vi "[ce low] Find All Min & Max of f(x).vi"(5 "# points":u32=1000, 6 "accuracy":dbl=1e-08 format="%.2e", 7 "VC Handle":T1=-1, 8 "error in":errorcluster, 9 "formula info":cluster{"formula":string, "x-variable":string}={"formula"="", "x-variable"="t"}, 10 "end":dbl=1.0 format="%.2f", 11 "start":dbl format="%.2f") -> (0 "error out":errorcluster, 2 "minima":cluster{"x":dbl[], "f(x)":dbl[]} {"f(x)" format="%.2f"; "x" format="%.2f"}, 3 "maxima":cluster{"x":dbl[], "f(x)":dbl[]} {"f(x)" format="%.2f"; "x" format="%.2f"})   [LabVIEW 2021]
doc: "::: CalcExpress Toolkit :::\nCopyright (c) 2000-2026 Konstantin Shifershteyn. All rights reserved."
uses:
  cetypes.llb/VarMan Variable Context Handle.ctl
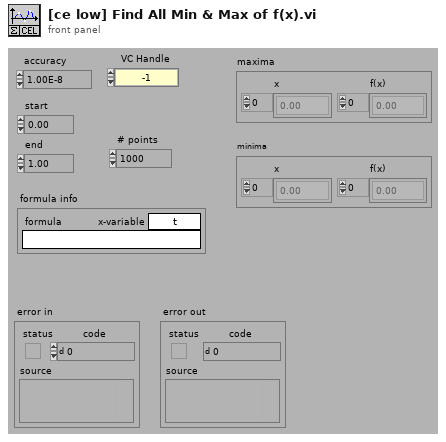
[diagram p1: front panel]
types:
  T1 = typedef "VarMan Variable Context Handle.ctl" = i32
  T2 = enum16{"create", "destroy", "set value", "get value"}
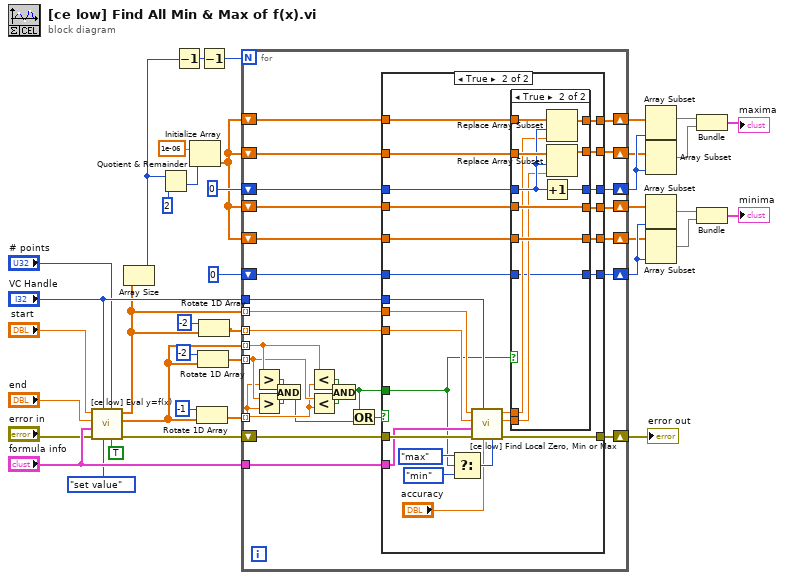
[diagram p0: block diagram]
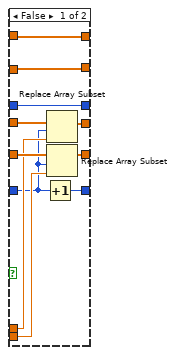
[diagram p3: hidden frame]
diagram:
  n1 = call "[ce low] Eval y=f(x).vi"("include end point"=TRUE ("extend range"), "# points"="# points", "vm cmd"=T2."set value", "VC Handle"="VC Handle", "error in"="error in", "formula info"="formula info", "end"="end", "start"="start") -> ("error out"=w33:errorcluster, "f(x)"=w5:dbl[], "x"=w2:dbl[])  [unwired: 1 out]
  n2 = Array Size(array=w2) -> (size(s)=w8:i32)
  n3 = Quotient & Remainder(x=w8, y=2) -> (floor(x/y)=w24:i32)  [unwired: 1 out]
  n4 = Decrement(x=w8) -> (x-1=w35:i32)
  n5 = Initialize Array(1e-06 ("accuracy"), w24) -> (w21:dbl[])
  n6 = Rotate 1D Array(1:w5, 2:-1) -> (0:w38:dbl[])
  n7 = Rotate 1D Array(1:w5, 2:-2) -> (0:w4:dbl[])
  n8 = Decrement(x=w35) -> (x-1=w7:i32)
  n9 = Rotate 1D Array(1:w2, 2:-2) -> (0:w36:dbl[])
  n10 = for {
    N: w7 -> [_]
    tunnel: w5 -> [w46] mode=indexing
    tunnel: w38 -> [w44] mode=indexing
    shift-right: [w66] -> w15
    shift-left: w21 -> [w67]
    shift-right: [w64] -> w14
    shift-left: w21 -> [w65]
    tunnel: w2 -> [w63] mode=indexing
    tunnel: w36 -> [w51] mode=indexing
    shift-right: [w40] -> w26
    shift-left: w33 -> [w62]
    tunnel: "formula info" -> [w61]
    shift-right: [w58] -> w16
    shift-left: w21 -> [w57]
    shift-right: [w60] -> w17
    shift-left: w21 -> [w59]
    tunnel: "VC Handle" -> [w56]
    shift-right: [w54] -> w18
    shift-left: 0 -> [w55]
    shift-right: [w52] -> w19
    shift-left: 0 -> [w53]
    tunnel: w4 -> [w45] mode=indexing
    n11 = Greater?(x=w46, y=w44) -> (0:w50:bool)
    n12 = Greater?(x=w45, y=w44) -> (0:w49:bool)
    n13 = And(x=w50, y=w49) -> (x .and. y?=w42:bool)
    n14 = Less?(x=w46, y=w44) -> (x < y?=w47:bool)
    n15 = Less?(x=w45, y=w44) -> (x < y?=w48:bool)
    n16 = And(x=w47, y=w48) -> (x .and. y?=w41:bool)
    n17 = Or(x=w41, y=w42) -> (x .or. y?=w43:bool)
    n18 = case shown="True" w43 {
      tunnel: w67 -> [w74 w99]
      tunnel: [w74 w98] -> w66
      tunnel: w65 -> [w73 w97]
      tunnel: [w73 w96] -> w64
      tunnel: w63 -> [_ w94]
      tunnel: w51 -> [_ w93]
      tunnel: w62 -> [w72 w95]
      tunnel: [w72 w92] -> w40
      tunnel: w61 -> [_ w91]
      tunnel: w57 -> [w71 w86]
      tunnel: [w71 w87] -> w58
      tunnel: w59 -> [w70 w88]
      tunnel: [w70 w89] -> w60
      tunnel: w56 -> [_ w84]
      tunnel: w55 -> [w69 w83]
      tunnel: [w69 w82] -> w54
      tunnel: w53 -> [w68 w81]
      tunnel: [w68 w80] -> w52
      tunnel: w41 -> [_ w75]
      frame False {
      }
      frame True {
        n19 = Select(t=enum16{"zero", "min", "max"}."max" ("find"), s=w75, f=enum16{"zero", "min", "max"}."min" ("find")) -> (s? t:f=w77:enum16{"zero", "min", "max"})
        n20 = call "[ce low] Find Local Zero, Min or Max.vi"("find"=w77, "accuracy"="accuracy", "VC Handle"=w84, "error in"=w95, "formula info"=w91, "end"=w93, "start"=w94) -> ("error out"=w92:errorcluster, "f(x)"=w85:dbl, "x"=w90:dbl)  [unwired: 2 in]
        n21 = case shown="True" w75 {
          tunnel: w99 -> [w107 w121]
          tunnel: [w104 w121] -> w98
          tunnel: w97 -> [w106 w120]
          tunnel: [w103 w120] -> w96
          tunnel: w90 -> [w101 w113]
          tunnel: w85 -> [w105 w112]
          tunnel: [w110 w118] -> w89
          tunnel: w88 -> [w110 w117]
          tunnel: [w109 w115] -> w87
          tunnel: w86 -> [w109 w116]
          tunnel: w83 -> [w108 w114]
          tunnel: [w108 w119] -> w82
          tunnel: w81 -> [w100 w111]
          tunnel: [w102 w111] -> w80
          frame False {
            n22 = Increment(x=w100) -> (x+1=w102:i32)
            n23 = Replace Array Subset(array=w107, new element=w101, index=w100) -> (w104:dbl[])
            n24 = Replace Array Subset(array=w106, new element=w105, index=w100) -> (w103:dbl[])
          }
          frame True {
            n25 = Increment(x=w114) -> (x+1=w119:i32)
            n26 = Replace Array Subset(array=w116, new element=w113, index=w114) -> (w115:dbl[])
            n27 = Replace Array Subset(array=w117, new element=w112, index=w114) -> (w118:dbl[])
          }
        }
      }
    }
  }
  "error out" <- w26
  n28 = Array Subset(array=w16, length=w18) -> (w13:dbl[])  [unwired: 1 in]
  n29 = Array Subset(array=w17, length=w18) -> (w12:dbl[])  [unwired: 1 in]
  n30 = Array Subset(array=w15, length=w19) -> (w11:dbl[])  [unwired: 1 in]
  n31 = Array Subset(array=w14, length=w19) -> (w10:dbl[])  [unwired: 1 in]
  n32 = Bundle(w13, w12) -> (→"maxima":cluster{dbl[], dbl[]})  [unwired: 1 in]
  n33 = Bundle(w11, w10) -> (→"minima":cluster{dbl[], dbl[]})  [unwired: 1 in]
